vi "Enemies_Init.vi"(0 "Tiles":u8[][](array[numeric]), 11 "error in":errorcluster) -> (4 "Enemies":T1(array[cluster]), 15 "error out":errorcluster)   [LabVIEW 2020, in "GH_Engine.lvlib"]
doc: "Builds the enemies of a room from its tiles: S spider (Kind 0), Z snake (1), K skull (2) at their start tiles, walking left or right (by the tile position), not climbing."
uses:
  GH_Engine.lvlib
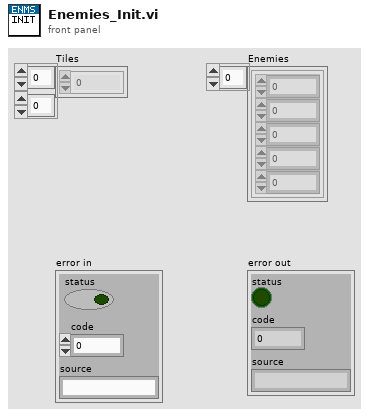
[diagram p1: front panel]
types:
  T1 = cluster{"Kind":i32, "X10":i32, "Y10":i32, "Dir":i32, "Mode":i32}[]
  T2 = cluster{"Kind":i32, "X10":i32, "Y10":i32, "Dir":i32, "Mode":i32}
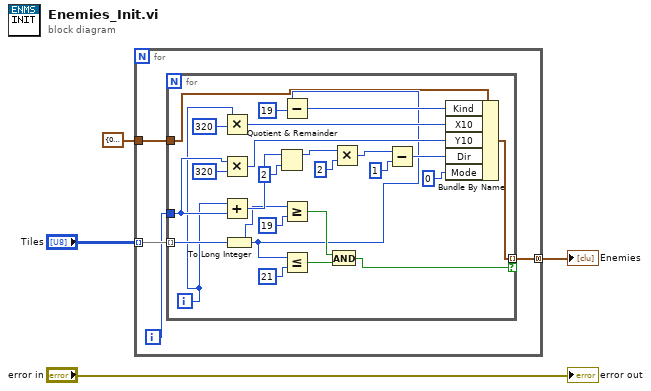
[diagram p0: block diagram]
diagram:
  n1 = for {
    tunnel: "Tiles" -> [w6] mode=indexing
    tunnel: T2 {"Kind"=0, "X10"=0, "Y10"=0, "Dir"=1, "Mode"=0} ("Enemy") -> [w7]
    tunnel: [w8] -> w4 mode=concatenating
    i -> [w5]
    n2 = for {
      tunnel: w5 -> [w12]
      tunnel: w6 -> [w10] mode=indexing
      tunnel: w7 -> [w11]
      tunnel: [w33] -> w8 mode=indexing if=w18
      i -> [w9]
      n3 = Multiply(x=w9, y=320) -> (x*y=w25:i32)
      n4 = Multiply(x=w12, y=320) -> (x*y=w27:i32)
      n5 = Add(x=w9, y=w12) -> (x+y=w19:i32)
      n6 = To Long Integer(number=w10) -> (32bit integer=w13:i32)
      n7 = Quotient & Remainder(x=w19, y=2) -> (x-y*floor(x/y)=w21:i32)  [unwired: 1 out]
      n8 = Subtract(x=w13, y=19) -> (x-y=w23:i32)
      n9 = Greater Or Equal?(x=w13, y=19) -> (x >= y?=w15:bool)
      n10 = Less Or Equal?(x=w13, y=21) -> (x <= y?=w17:bool)
      n11 = And(x=w15, y=w17) -> (x .and. y?=w18:bool)
      n12 = Multiply(x=w21, y=2) -> (x*y=w29:i32)
      n13 = Subtract(x=w29, y=1) -> (x-y=w31:i32)
      n14 = Bundle By Name(cluster=w11, "Kind"=w23, "X10"=w25, "Y10"=w27, "Dir"=w31, "Mode"=0) -> (w33:T2)
    }
  }
  "Enemies" <- w4
  "error out" <- "error in"
